vi "Get Status.vi"(8 "error in (no error)":errorcluster, 11 "bt_System in":refnum<class "bt_System.lvclass">) -> (0 "error out":errorcluster, 2 "Status":T1, 3 "bt_System out":refnum<class "bt_System.lvclass">)   [LabVIEW 2021, in "BT.lvlib" / "bt_System.lvclass"]
uses:
  bt_System.lvclass
  Support/Nodes/abs_Node/Status.ctl
  bt_System.lvclass/bt_System.ctl
  Support/Nodes/abs_Node/bt_Node.lvclass
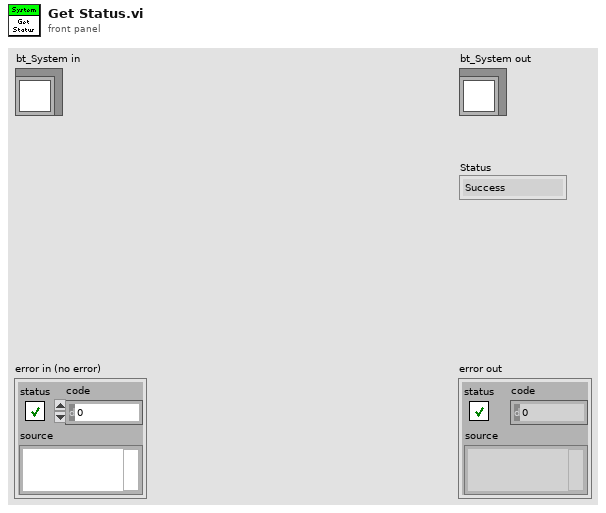
[diagram p1: front panel]
types:
  T1 = typedef "BT.lvlib/bt_Node.lvclass/Status.ctl" = enum16{"Success", "Failure", "Running"}
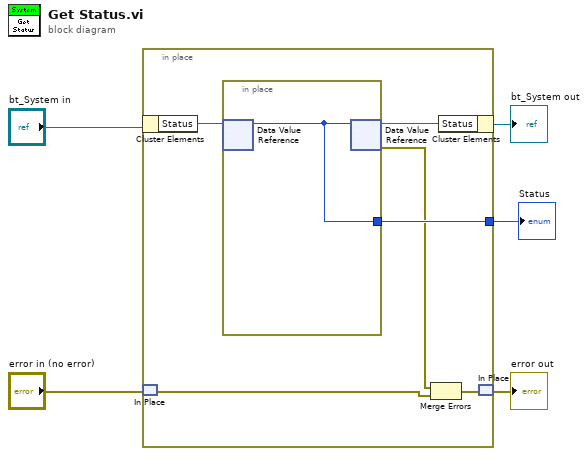
[diagram p0: block diagram]
diagram:
  n1 = in-place {
    in-place-border: [w10] -> w3
    n2 = in-place-cluster #1("bt_System in") -> ("Status"=w11:refnum<data-value>)
    n3 = in-place-match #2("error in (no error)") -> (w8:errorcluster)
    n4 = in-place {
      in-place-border: [w12] -> w10
      n5 = in-place-dvr #3(w11) -> (w12:T1)  [unwired: 1 out]
      n6 = in-place-dvr #3(w12) -> (w9:refnum<data-value>, w7:errorcluster)
    }
    n7 = Merge Errors(w7, w8) -> (w6:errorcluster)
    n8 = in-place-cluster #1("Status"=w9) -> (→"bt_System out":refnum<class "bt_System.lvclass">)
    n9 = in-place-match #2(w6) -> (→"error out":errorcluster)
  }
  "Status" <- w3
